vi "Reset Results.vi"(8 "error in":errorcluster, 11 "Sequence Executor in":refnum<class "Sequence Executor.lvclass">) -> (0 "error out":errorcluster, 3 "Sequence Executor out":refnum<class "Sequence Executor.lvclass">)   [LabVIEW 2026, in "Sequence Executor.lvclass"]
doc: "PRIVATE. Rebuilds Results from Sequence.steps: one Step Result per step with result NOT RUN, empty reason, zero numbers."
uses:
  Sequence Executor.lvclass
  Sequence Executor.lvclass/Sequence Executor.ctl
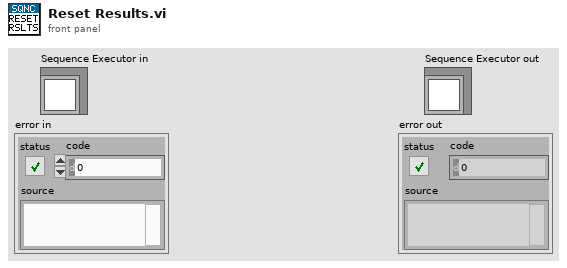
[diagram p1: front panel]
types:
  T1 = cluster{"step_no":i32, "step_name":string, "result":string, "reason":string, "measured":dbl, "target":dbl, "duration_ms":dbl}
  T2 = typedef "Sequence File.ctl" = cluster{"sequence_id":string, "description":string, "rig_config":string, "steps":T3[]}
  T3 = typedef "Step Config.ctl" = cluster{"step_no":i32, "step_name":string, "command_type":string, "setpoints":T4[], "conditions":T5[], "dwell_time_ms":i32, "timeout_ms":i32, "expected_result":string}
  T4 = typedef "Channel Value.ctl" = cluster{"channel":string, "value":dbl}
  T5 = typedef "Condition.ctl" = cluster{"channel":string, "target":dbl, "tolerance":dbl}
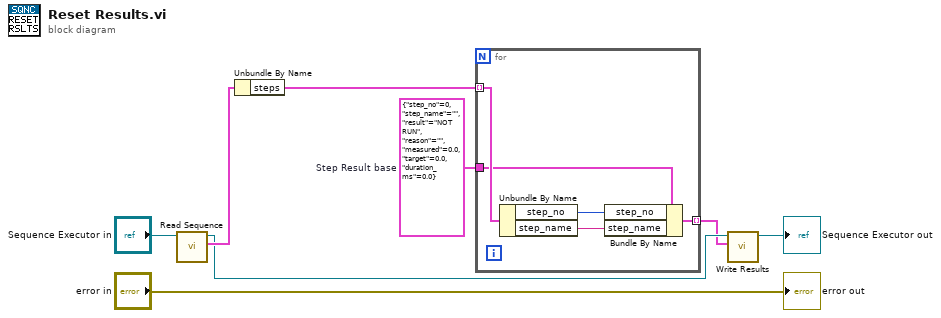
[diagram p0: block diagram]
diagram:
  w5 = T1 {"step_no"=0, "step_name"="", "result"="NOT RUN", "reason"="", "measured"=0.0, "target"=0.0, "duration_ms"=0.0}  # Step Result base
  n1 = call "Read Sequence.vi"("Sequence Executor in"="Sequence Executor in") -> ("Sequence File"=w7:T2, "Sequence Executor out"=w4:refnum<class "Sequence Executor.lvclass">)  [unwired: 8 in, 1 out]
  n2 = Unbundle By Name(w7) -> ("steps"=w6:T3[])
  n3 = for {
    tunnel: w6 -> [w13] mode=indexing
    tunnel: w5 -> [w10]
    tunnel: [w9] -> w3 mode=indexing
    n4 = Unbundle By Name(w13) -> ("step_no"=w12:i32, "step_name"=w11:string)
    n5 = Bundle By Name(cluster=w10, "step_no"=w12, "step_name"=w11) -> (w9:T1)
  }
  n6 = call "Write Results.vi"("Results"=w3, "Sequence Executor in"=w4) -> ("Sequence Executor out"=→"Sequence Executor out":refnum<class "Sequence Executor.lvclass">)  [unwired: 8 in, 1 out]
  "error out" <- "error in"
